vi "FuncVI-Derivate.vi"(5 "InstanceRef":T2, 9 "arg list":T1[](array[typedef]) {"num" format="%.2f"}) -> (0 "error out":bool, 3 "result":T1 {"num" format="%.2f"})   [LabVIEW 2021]
doc: "::: CalcExpress Toolkit :::\nCopyright (c) 2000-2026 Konstantin Shifershteyn. All rights reserved."
uses:
  cetypes.llb/CalcExpress Function Argument Info.ctl
  cetypes.llb/CalcExpress Instance RefNum.ctl
  <vilib>/Analysis/2dsp.llb/Derivative x(t).vi
  <vilib>/Analysis/NI_AALPro.lvlib
panel:
  in  "max arg num":i32=4
  in  "min arg num":i32=1
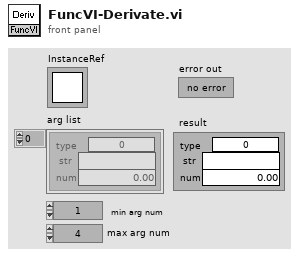
[diagram p1: front panel]
types:
  T1 = typedef "CalcExpress Function Argument Info.ctl" = cluster{"type":u32, "str":string, "num":dbl}
  T2 = typedef "CalcExpress Instance RefNum.ctl" = refnum<k1>
  T3 = enum8{"String", "DBL Number", "identifier", "1D Array of DBL", "2D Array of DBL", "CDB Number", "1D Array of CDB", "2D Array of CDB", "1D Array of String", "2D Array of String", "Unknown data type"}
  T4 = cluster{"index":i32, "type":enum8{"String", "DBL Number", "identifier", "1D Array of DBL", "2D Array of DBL", "CDB Number", "1D Array of CDB", "2D Array of CDB", "Unknown data type"}, "default num":dbl, "default str":string}[]
  T5 = cluster{"num list[0]":dbl, "num list[1]":dbl, "num list[2]":dbl, "num list[3]":dbl}
  T6 = cluster{"type":enum8{"String", "DBL Number", "identifier", "1D Array of DBL", "2D Array of DBL", "CDB Number", "1D Array of CDB", "2D Array of CDB", "1D Array of String", "2D Array of String", "Unknown data type"}, "data string":string, dbl}
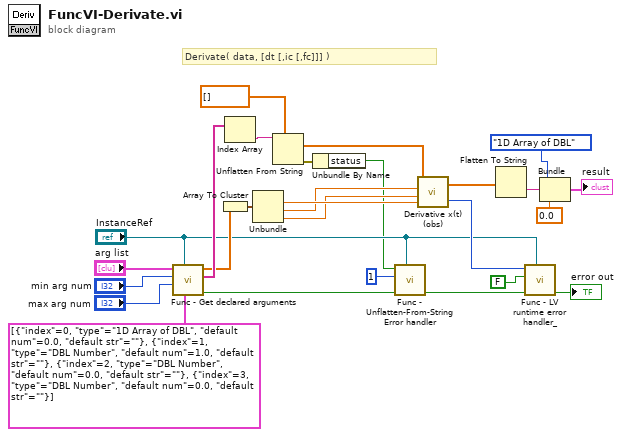
[diagram p0: block diagram]
diagram:
  # "Derivate( data, [dt [,ic [,fc]]] )"
  n1 = call "Func - Get declared arguments.vi"("arg descriptors"=T4 [{"index"=0, "type"=enum."1D Array of DBL", "default num"=0.0, "default str"=""}, {"index"=1, "type"=enum."DBL Number", "default num"=1.0, "default str"=""}, {"index"=2, "type"=enum."DBL Number", "default num"=0.0, "default str"=""}, {"index"=3, "type"=enum."DBL Number", "default num"=0.0, "default str"=""}] ("args descriptors"), "InstanceRef"="InstanceRef", "max arg num"="max arg num", "min arg num"="min arg num", "arg list"="arg list") -> ("error out"=w8:bool, "str list"=w24:string[], "num list"=w14:dbl[])  [unwired: 3 in, 1 out]
  n2 = Array To Cluster(array=w14) -> (cluster=w13:T5)
  n3 = Index Array(array=w24) -> (element=w23:string)  [unwired: 1 in]
  n4 = Unbundle(w13) -> ("num list[1]"=w12:dbl, "num list[2]"=w11:dbl, "num list[3]"=w10:dbl)  [unwired: 1 out]
  n5 = Unflatten From String(type=dbl[] [], binary string=w23) -> (value=w15:dbl[], error out=w1:errorcluster)  [unwired: 3 in, 1 out]
  n6 = Unbundle By Name(w1) -> ("status"=w5:bool)
  n7 = call "Func - Unflatten-From-String Error handler.vi"("InstanceRef"="InstanceRef", "error in"=w8, "argument number"=1, "Unflatten Error status"=w5) -> ("error out"=w7:bool)  [unwired: 5 in]
  n8 = call <vilib>:"Derivative x(t) (obs).vi"("dt"=w12, "final condition"=w10, "initial condition"=w11, "X"=w15) -> ("error"=w17:i32, "dX/dt"=w21:dbl[])
  n9 = Flatten To String(anything=w21) -> (data string=w19:string)  [unwired: 3 in, 2 out]
  n10 = call "Func - LV runtime error handler_.vi"("InstanceRef"="InstanceRef", "error in"=w7, "Gen CE error?"=FALSE, "LabVIEW error code"=w17) -> ("error out"=→"error out":bool)  [unwired: 7 in]
  n11 = Bundle("type"=T3."1D Array of DBL", "data string"=w19, 0.0) -> (→"result":T6)  [unwired: 1 in]
